vi "OwnOop20261013_CreateChild.vi"() -> ()   [LabVIEW 2024]
uses:
  <resource>/Framework/Providers/AddClass/Add Class.lvlib
panel:
  out "error out":errorcluster caption="错误输出"
  in  "Class Path":path
  in  "Parent Path":path
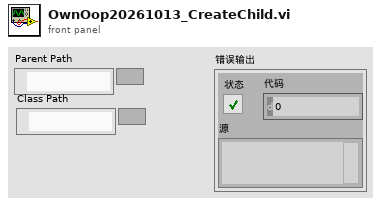
[diagram p1: front panel]
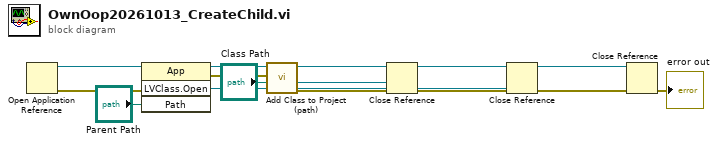
[diagram p0: block diagram]
diagram:
  n1 = Open Application Reference() -> (0:w9:errorcluster, 3:w11:refnum<vi>)  [unwired: 4 in]
  n2 = invoke class="App" method="LVClass.Open"(reference=w11, error in=w9, "Path"="Parent Path") -> (error out=w6:errorcluster, "LVClass.Open"=w7:refnum<vi>)  [unwired: 1 in, 2 out]
  n3 = call <resource>:"Add Class to Project (path).vi"("Parent Class"=w7, "Application"=w11, "error in"=w6, "Class Path"="Class Path") -> ("error out"=w4:errorcluster, "Class"=w5:refnum<vi>)  [unwired: 6 in]
  n4 = Close Reference(reference=w5, error in (no error)=w4) -> (error out=w3:errorcluster)
  n5 = Close Reference(reference=w7, error in (no error)=w3) -> (error out=w2:errorcluster)
  n6 = Close Reference(reference=w11, error in (no error)=w2) -> (error out=→"error out":errorcluster)
